vi "CIF Publish Raw.vi"(8 "error in (no error)":errorcluster, 9 "Timeout ms":u32, 10 "Data In":u8[](array[numeric]), 11 "Publisher Reference":T2 {"refnum" format="%.0x"}) -> (0 "error out":errorcluster, 1 "Timeout":bool, 2 "Data Out":u8[](array[numeric]), 4 "CIF Publisher Stats":T1)   [LabVIEW 2021, in "Iceoryx.lvlib"]
doc: "Publish to an iceoryx CIF pcap queue with a manually provided CIF header. This is normally used if the payload is being received as a \"black box\" message such as a TCP stream from another machine. This will write to both publisher queues if created. If there is a backpressure queue with a subscriber attached it can block this VI and it will timeout. On timeout no data will be written to either queue. \n\n<B>Data In:</B> Flattened CIF header and the flattened PCAP formatted data of the correct Link Type. Note the length and counter values in the header will still be updated automatically. \n<B>Timeout:</B> Timeout in ms if there is a backpressure queue. \n<B>CIF Publish Advanced:</B> Allows copying a subset of the Data In array. This is useful for variable size payloads where a larger buffer is allocated but only the valid data should be passed."
uses:
  Iceoryx.lvlib
  Refnum/Typedef/CIF Publisher Refnum.ctl
  typedef/CIF Pcap Publisher Stats.ctl
  SubVIs/Convert Error Core.vi
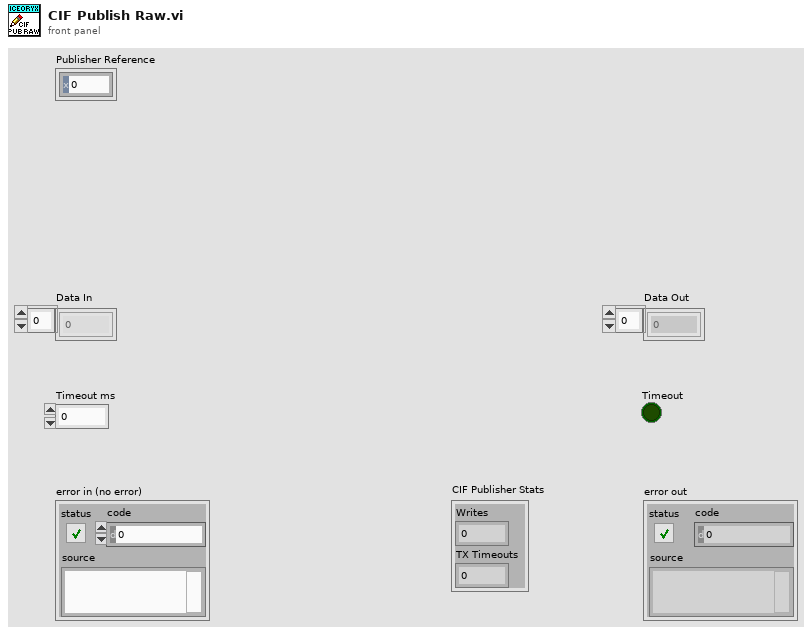
[diagram p1: front panel]
types:
  T1 = typedef "Iceoryx.lvlib/CIF Pcap Publisher Stats.ctl" = cluster{"Writes":u64, "TX Timeouts":u64}
  T2 = typedef "Iceoryx.lvlib/CIF Publisher Refnum.ctl" = cluster{"refnum":u64, "CIF Pub":enum8{"cifpub"}}
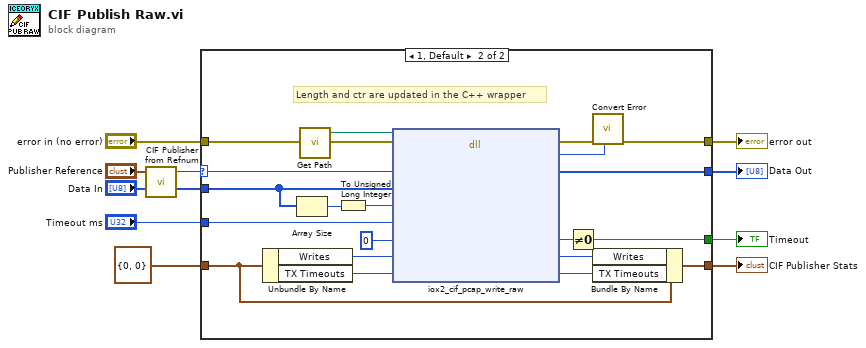
[diagram p0: block diagram]
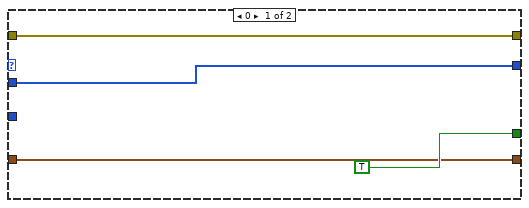
[diagram p2: hidden frame]
diagram:
  n1 = call "CIF Publisher from Refnum.vi"("CIF Publisher Refnum"="Publisher Reference") -> ("CIF Publisher U64"=w1:u64)  [unwired: 4 in]
  n2 = case shown="1, Default" w1 {
    selector: w1 -> [_ w29]
    tunnel: "error in (no error)" -> [w14 w34]
    tunnel: [w14 w30] -> w9
    tunnel: "Timeout ms" -> [_ w28]
    tunnel: [TRUE w26] -> w6
    tunnel: "Data In" -> [w12 w15]
    tunnel: [w12 w24] -> w4
    tunnel: [w11 w21] -> w3
    tunnel: T1 {"Writes"=0, "TX Timeouts"=0} ("CIF Publisher Stats") -> [w11 w20]
    frame 0 {
    }
    frame 1, Default {
      # "Length and ctr are updated in the C++ wrapper"
      n3 = Unbundle By Name(w20) -> ("Writes"=w19:u64, "TX Timeouts"=w18:u64)
      n4 = Array Size(array=w15) -> (size(s)=w17:i32)
      n5 = call "Get Path.vi"() -> ("libiox2_cif path"=w33:path)  [unwired: 4 in]
      n6 = To Unsigned Long Integer(number=w17) -> (unsigned 32bit integer=w16:u32)
      n7 = dll-call lib="D:/dev/iceoryx2_lvwrapper/dist/iox2_cif.dll" fn="iox2_cif_pcap_write_raw"(path in=w33, error in=w34, "writer"=w29, "sample"=w15, "length"=w16, "timeout_ms"=w28, "timed_out"=0, "samples"=w19, "timeouts"=w18) -> (error out=w32:errorcluster, "return type"=w31:i32, "sample"=w24:u8[], "timed_out"=w27:i32, "samples"=w22:u64, "timeouts"=w23:u64)  [unwired: 4 in, 1 out]
      n8 = Not Equal To 0?(x=w27) -> (x != 0?=w26:bool)
      n9 = call "Convert Error.vi"("return type"=w31, "error in (no error)"=w32) -> ("error out"=w30:errorcluster)  [unwired: 9 in]
      n10 = Bundle By Name(cluster=w20, "Writes"=w22, "TX Timeouts"=w23) -> (w21:T1)
    }
  }
  "error out" <- w9
  "Timeout" <- w6
  "Data Out" <- w4
  "CIF Publisher Stats" <- w3
